vi "Shot_timing.vi"(0 "valve_delay":dbl=150.0, 1 "gate_len_ms":dbl=20.0, 2 "start_delay_ms":dbl=150.0, 3 "rate":dbl=1000.0, 5 "valve_pulse_ms":dbl=50.0, 7 "camera_pulse_ms":dbl=50.0, 9 "flow_lag_ms":dbl=30.0, 11 "pre_flow_ms":dbl=10.0, 12 "trigger_gap_ms":dbl=10.0, 13 "capture_time_ms":dbl=200.0, 14 "tail_ms":dbl=50.0) -> (4 "gate_start_ms":dbl, 6 "camera_delay":dbl, 8 "pulse_length_ms":dbl, 10 "fail_code":i32, 15 "Timing_msg":string)   [LabVIEW 2025]
panel:
  out "Timing_OK":bool
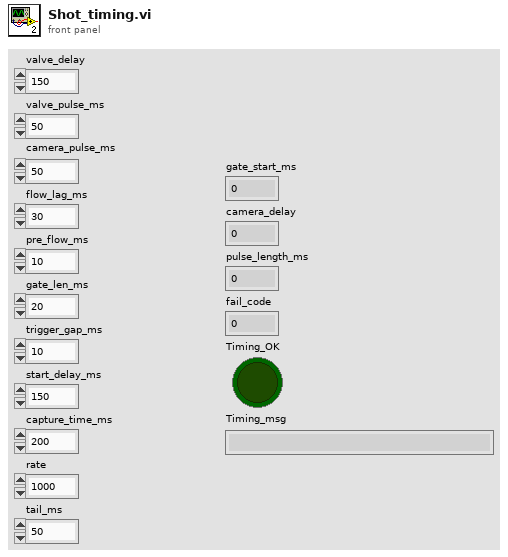
[diagram p1: front panel]
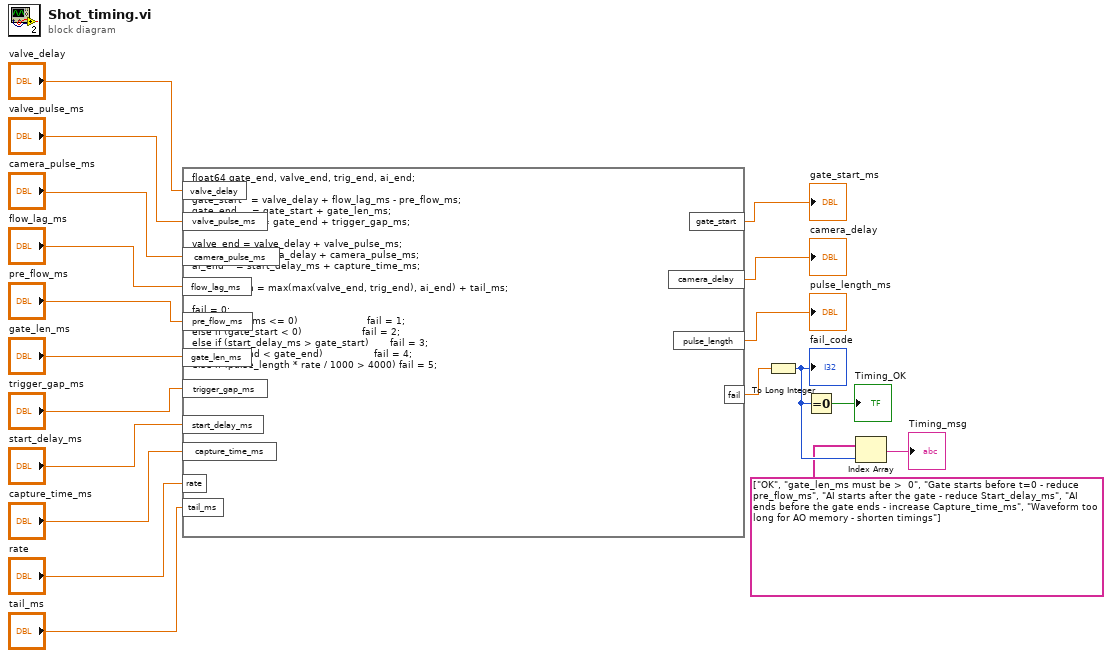
[diagram p0: block diagram]
diagram:
  n1 = formula code="float64 gate_end, valve_end, trig_end, ai_end;\n\ngate_start   = valve_delay + flow_lag_ms - pre_flow_ms;\ngate_end     = gate_start + gate_len_ms;\ncamera_delay = gate_end + trigger_gap_ms;\n\nvalve_end = valve_delay + valve_pulse_ms;\ntrig_end  = camera_delay + camera_pulse_ms;\nai_end    = start_delay_ms + capture_time_ms;\n\npulse_length = max(max(valve_end, trig_end), ai_end) + tail_ms;\n\nfail = 0;\nif (gate_len_ms <= 0)                       fail = 1;\nelse if (gate_start < 0)                    fail = 2;\nelse if (start_delay_ms > gate_start)       fail = 3;\nelse if (ai_end < gate_end)                 fail = 4;\nelse if (pulse_length * rate / 1000 > 4000) fail = 5;"("valve_pulse_ms"="valve_pulse_ms", "camera_pulse_ms"="camera_pulse_ms", "flow_lag_ms"="flow_lag_ms", "valve_delay"="valve_delay", "pre_flow_ms"="pre_flow_ms", "gate_len_ms"="gate_len_ms", "trigger_gap_ms"="trigger_gap_ms", "start_delay_ms"="start_delay_ms", "capture_time_ms"="capture_time_ms", "rate"="rate", "tail_ms"="tail_ms") -> ("gate_start"=→"gate_start_ms":dbl, "camera_delay"=→"camera_delay":dbl, "pulse_length"=→"pulse_length_ms":dbl, "fail"=w5:dbl)
  n2 = To Long Integer(number=w5) -> (32bit integer=w3:i32)
  "fail_code" <- w3
  n3 = Equal To 0?(x=w3) -> (x = 0?=→"Timing_OK":bool)
  n4 = Index Array(array=string[] ["OK", "gate_len_ms must be >  0", "Gate starts before t=0 - reduce pre_flow_ms", "AI starts after the gate - reduce Start_delay_ms", "AI ends before the gate ends - increase Capture_time_ms", "Waveform too long for AO memory - shorten timings"], index=w3) -> (element=→"Timing_msg":string)
